vi "FunctionCallToJsonRpcRequestCluster.vi"(8 "error in (no error)":errorcluster, 10 "FunctionCall":T2) -> (0 "error out":errorcluster, 2 "JsonRPCHttpRequestBody":T1)   [LabVIEW 2017]
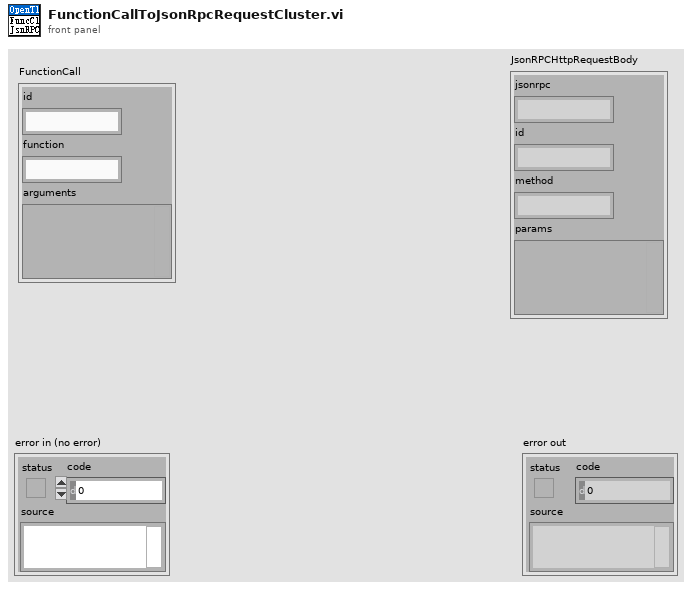
[diagram p1: front panel]
types:
  T1 = cluster{"jsonrpc":string, "id":string, "method":string, "params":variant}
  T2 = cluster{"id":string, "function":string, "arguments":variant}
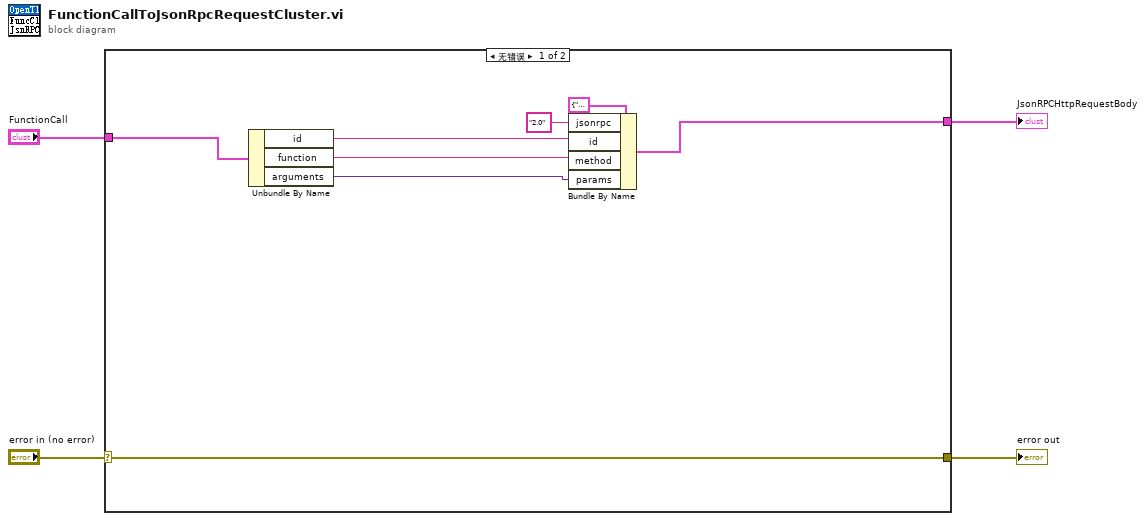
[diagram p0: block diagram]
diagram:
  n1 = case shown="无错误" "error in (no error)" {
    selector: "error in (no error)" -> [w5 w13]
    tunnel: [w5 w13] -> w3
    tunnel: "FunctionCall" -> [w11 _]
    tunnel: [w6 _] -> w1
    frame No Error {
      n2 = Unbundle By Name(w11) -> ("id"=w10:string, "function"=w8:string, "arguments"=w7:variant)
      n3 = Bundle By Name(cluster=T1 {"jsonrpc"="", "id"="", "method"="", "params"=variant} ("JsonRPCHttpRequestBody"), "jsonrpc"="2.0", "id"=w10, "method"=w8, "params"=w7) -> (w6:T1)
    }
    frame Error {
    }
  }
  "error out" <- w3
  "JsonRPCHttpRequestBody" <- w1
